vi "SUP_Camera_Epoch.vi"(5 "error in (no error)":errorcluster, 6 "Image":T1, 7 "valeur de l'horloge en ms 3":u32, 8 "SetupOK":bool, 9 "valeur de l'horloge en ms 2":u32, 10 "temps actuel":timestamp, 11 "valeur de l'horloge en ms":u32) -> (0 "valid_for_run":bool, 1 "channel_out":u32, 2 "capture":timestamp, 3 "error in (no error) 2":errorcluster, 4 "Image 2":T1)   [LabVIEW 2012]
uses:
  <vilib>/vision/Image Controls.llb/IMAQ Image.ctl
panel:
  in  "temps actuel 3":timestamp
  out "error in (no error) 3":errorcluster
  in  "temps actuel 2":timestamp
  out "Image Pixels (I16)":i16[][](array[numeric])
  out "Image Pixels (U8)":u8[][](array[numeric])
  out "error out":errorcluster
  out "Image Pixels (Float)":sgl[][](array[numeric]) format="%.2f"
  out "Image Pixels (U16)":u16[][](array[numeric])
  in  "Optional Rectangle":i32[](array[numeric])
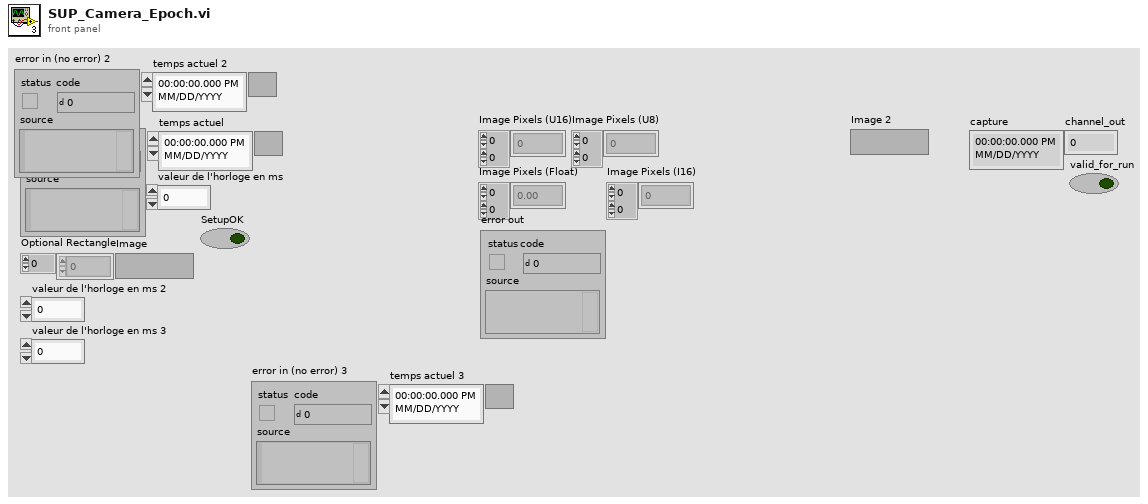
[diagram p1: front panel]
types:
  T1 = typedef "IMAQ Image.ctl" = refnum<image>
  T2 = cluster{"temps actuel":timestamp, "temps actuel 3":timestamp, "valeur de l'horloge en ms 2":u32, bool}
  T3 = cluster{"temps actuel":timestamp, "temps actuel 3":timestamp, "valeur de l'horloge en ms 2":u32, "SetupOK":bool}
  T4 = cluster{"temps actuel":timestamp, "temps actuel":timestamp, "valeur de l'horloge en ms 2":u32, bool}
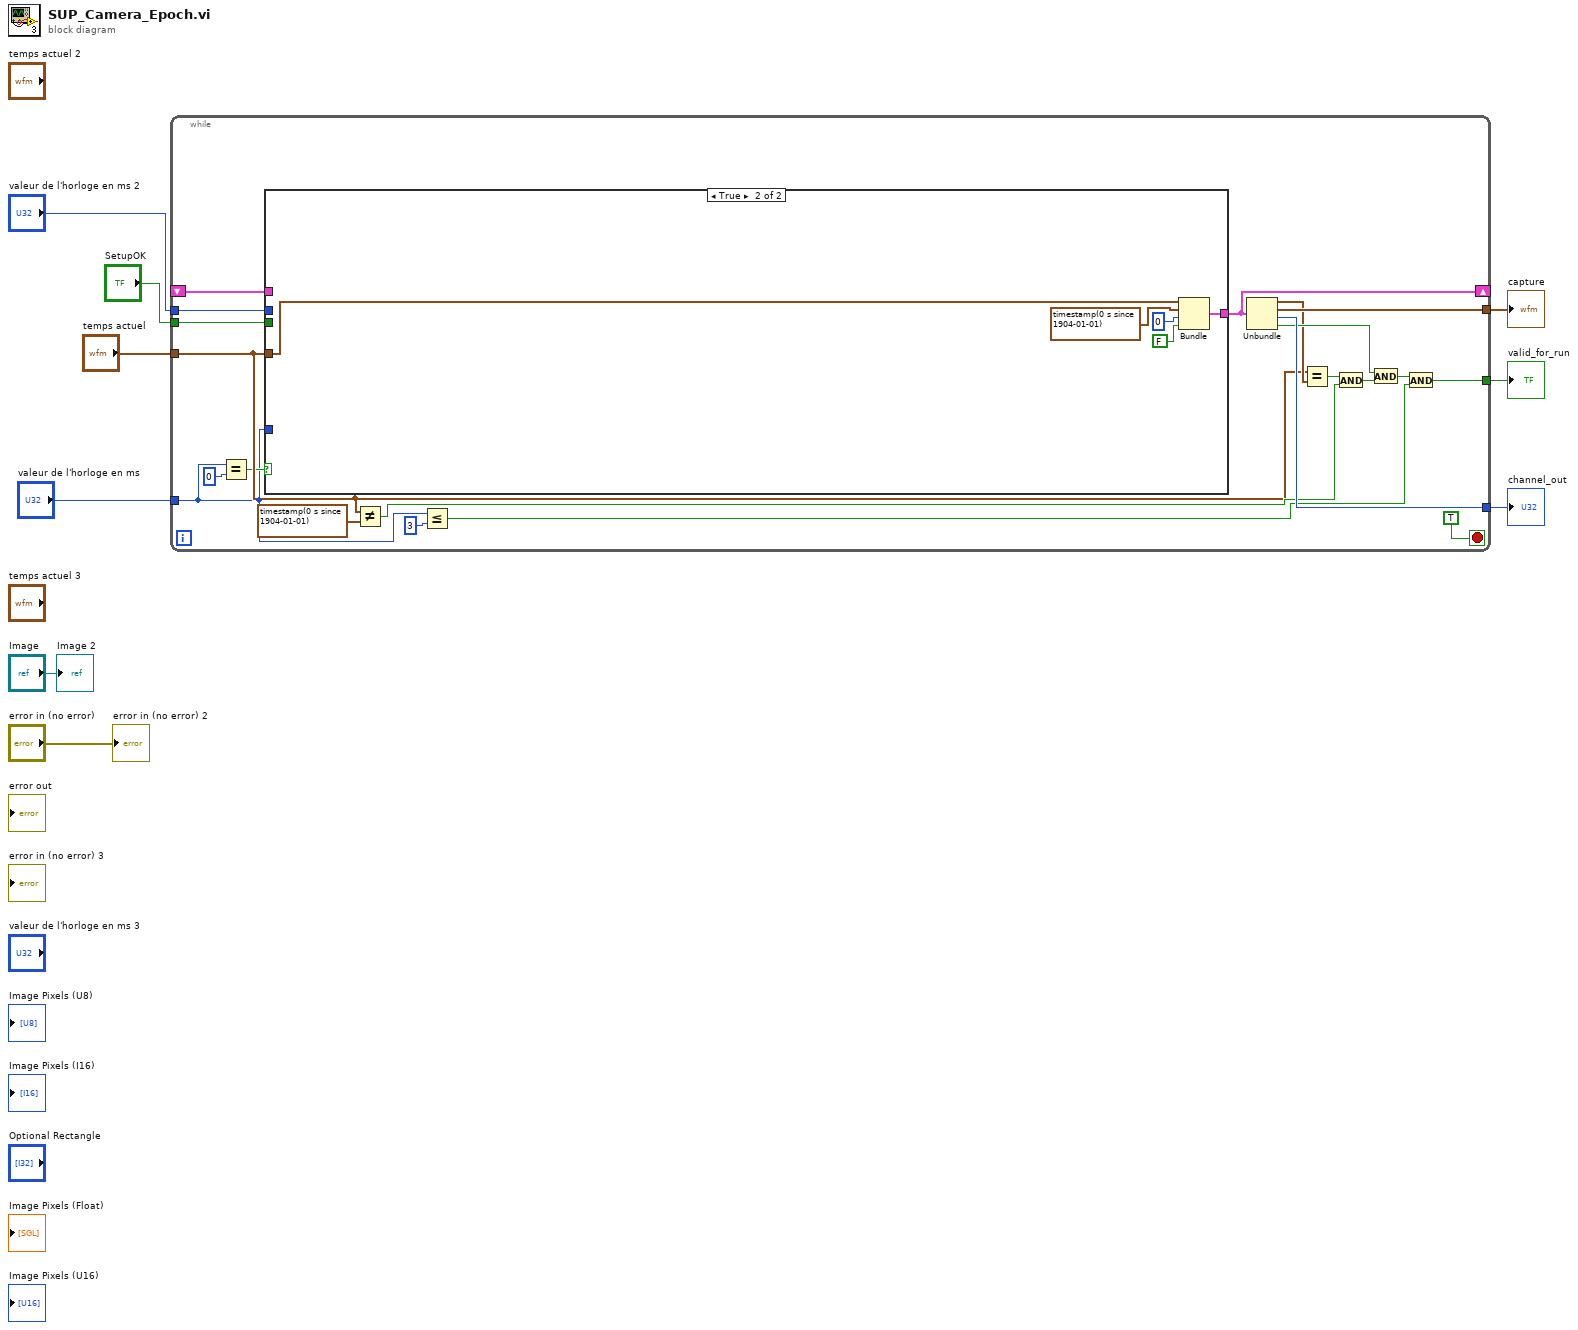
[diagram p0: block diagram]
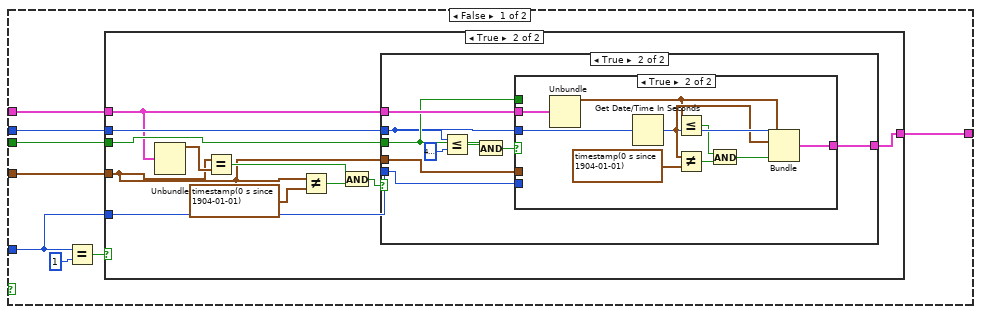
[diagram p2: hidden frame]
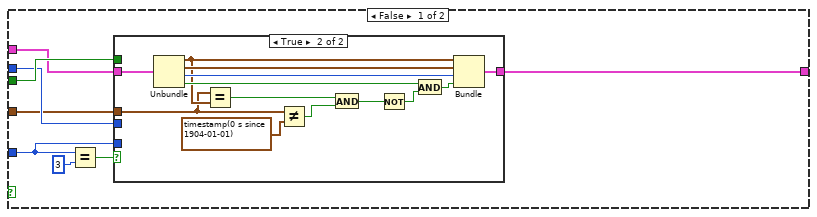
[diagram p3: hidden frame]
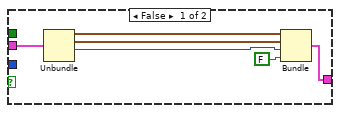
[diagram p6: hidden frame]
diagram:
  n1 = while {
    shift-right: [w18] -> _
    shift-left: _ -> [w14]
    tunnel: "valeur de l'horloge en ms" -> [w11]
    tunnel: "temps actuel" -> [w15]
    tunnel: "valeur de l'horloge en ms 2" -> [w16]
    tunnel: "SetupOK" -> [w17]
    tunnel: [w28] -> w5
    tunnel: [w29] -> w6
    tunnel: [w30] -> w7
    stop <- TRUE stop-if-true
    n2 = Equal?(x=w11, y=u32 0 ("valeur de l'horloge en ms 2")) -> (x = y?=w13:bool)
    n3 = case shown="True" w13 {
      tunnel: w14 -> [w34 _]
      tunnel: w11 -> [w31 _]
      tunnel: w15 -> [w35 w97]
      tunnel: w16 -> [w36 _]
      tunnel: w17 -> [w37 _]
      tunnel: [w38 w101] -> w18
      frame False {
        n4 = Equal?(x=w31, y=u32 1 ("valeur de l'horloge en ms 2")) -> (x = y?=w33:bool)
        n5 = case shown="True" w33 {
          tunnel: w34 -> [w42 w61]
          tunnel: w31 -> [w39 w68]
          tunnel: w35 -> [w43 w62]
          tunnel: w36 -> [w44 w69]
          tunnel: w37 -> [w45 w70]
          tunnel: [w46 w71] -> w38
          frame False {
            n6 = Equal?(x=w39, y=u32 3 ("valeur de l'horloge en ms 2")) -> (x = y?=w41:bool)
            n7 = case shown="True" w41 {
              tunnel: w42 -> [w47 w48]
              tunnel: w39 -> [_ _]
              tunnel: w43 -> [_ w49]
              tunnel: w44 -> [_ _]
              tunnel: w45 -> [_ _]
              tunnel: [w47 w60] -> w46
              frame False {
              }
              frame True {
                n8 = Unbundle(w48) -> ("temps actuel"=w50:timestamp, "temps actuel 3"=w57:timestamp, "valeur de l'horloge en ms 2"=w58:u32, "SetupOK"=w55:bool)
                n9 = Equal?(x=w49, y=w50) -> (x = y?=w52:bool)
                n10 = Not Equal?(x=w49, y=timestamp(0 s since 1904-01-01) ("temps actuel 3")) -> (x != y?=w53:bool)
                n11 = And(x=w52, y=w53) -> (x .and. y?=w54:bool)
                n12 = Not(x=w54) -> (.not. x?=w56:bool)
                n13 = And(x=w55, y=w56) -> (x .and. y?=w59:bool)
                n14 = Bundle("temps actuel"=w50, "temps actuel 3"=w57, "valeur de l'horloge en ms 2"=w58, w59) -> (w60:T2)  [unwired: 1 in]
              }
            }
          }
          frame True {
            n15 = Unbundle(w61) -> ("temps actuel"=w63:timestamp)  [unwired: 3 out]
            n16 = Equal?(x=w62, y=w63) -> (x = y?=w65:bool)
            n17 = Not Equal?(x=w62, y=timestamp(0 s since 1904-01-01) ("temps actuel 3")) -> (x != y?=w66:bool)
            n18 = And(x=w65, y=w66) -> (x .and. y?=w67:bool)
            n19 = case shown="True" w67 {
              tunnel: w61 -> [w72 w78]
              tunnel: w68 -> [_ w79]
              tunnel: w62 -> [_ w80]
              tunnel: w69 -> [_ w73]
              tunnel: w70 -> [_ w76]
              tunnel: [w72 w81] -> w71
              frame False {
              }
              frame True {
                n20 = Less Or Equal?(x=w73, y=u32 4294967295 ("valeur de l'horloge en ms 2")) -> (x <= y?=w75:bool)
                n21 = And(x=w75, y=w76) -> (x .and. y?=w77:bool)
                n22 = case shown="True" w77 {
                  tunnel: w78 -> [w82 w88]
                  tunnel: w79 -> [_ _]
                  tunnel: w80 -> [_ _]
                  tunnel: w73 -> [_ w94]
                  tunnel: w76 -> [_ _]
                  tunnel: [w87 w96] -> w81
                  frame False {
                    n23 = Unbundle(w82) -> ("temps actuel"=w83:timestamp, "temps actuel 3"=w84:timestamp, "valeur de l'horloge en ms 2"=w85:u32)  [unwired: 1 out]
                    n24 = Bundle("temps actuel"=w83, "temps actuel 3"=w84, "valeur de l'horloge en ms 2"=w85, "SetupOK"=FALSE) -> (w87:T3)  [unwired: 1 in]
                  }
                  frame True {
                    n25 = Unbundle(w88) -> ("temps actuel"=w89:timestamp)  [unwired: 3 out]
                    n26 = Get Date/Time In Seconds() -> (seconds since 1Jan1904=w90:timestamp)
                    n27 = Less Or Equal?(x=w89, y=w90) -> (x <= y?=w92:bool)
                    n28 = Not Equal?(x=w90, y=timestamp(0 s since 1904-01-01) ("temps actuel 3")) -> (x != y?=w93:bool)
                    n29 = And(x=w92, y=w93) -> (x .and. y?=w95:bool)
                    n30 = Bundle("temps actuel"=w89, "temps actuel"=w90, "valeur de l'horloge en ms 2"=w94, w95) -> (w96:T4)  [unwired: 1 in]
                  }
                }
              }
            }
          }
        }
      }
      frame True {
        n31 = Bundle("temps actuel"=w97, "temps actuel 3"=timestamp(0 s since 1904-01-01), "valeur de l'horloge en ms 2"=u32 0, "SetupOK"=FALSE) -> (w101:T3)  [unwired: 1 in]
      }
    }
    n32 = Not Equal?(x=w15, y=timestamp(0 s since 1904-01-01) ("temps actuel 3")) -> (x != y?=w22:bool)
    n33 = Less Or Equal?(x=w11, y=u32 3 ("valeur de l'horloge en ms 2")) -> (x <= y?=w27:bool)
    n34 = Unbundle(w18) -> ("temps actuel"=w19:timestamp, "temps actuel 3"=w28:timestamp, "valeur de l'horloge en ms 2"=w29:u32, "SetupOK"=w23:bool)
    n35 = Equal?(x=w15, y=w19) -> (x = y?=w21:bool)
    n36 = And(x=w21, y=w22) -> (x .and. y?=w24:bool)
    n37 = And(x=w23, y=w24) -> (x .and. y?=w26:bool)
    n38 = And(x=w26, y=w27) -> (x .and. y?=w30:bool)
  }
  "capture" <- w5
  "channel_out" <- w6
  "valid_for_run" <- w7
  "error in (no error) 2" <- "error in (no error)"
  "Image 2" <- "Image"
